vi "CONFIG PRES+TEMP+REG V115.vi"() -> ()   [LabVIEW 2022 SP3]
uses:
  Pressions/Gestion grappe/TypeDef_Seuil Jauge Pression_CN.ctl
  Enum/Enum conf 1.ctl
  Variables globales/Variable glob Edwards.vi
  Variables globales/Variable glob Th.vi
  Variables globales/Variable glob Pt.vi
  Variables globales/Variable glob Leybold.vi
  Variables globales/Variable glob Keller.vi
  Variables globales/Variable glob generale.vi
  Variables globales/Variables glob EUROTHERM.vi
  Variables globales/Variable globale compteurs.vi
  Variables globales/Variable glob mails.vi
  <vilib>/Utility/config.llb/NI_LVConfig.lvlib
panel:
  in  "annuler":bool
  out "Dossier DATA local :":path
  in  "Commande onglet":T1(tab)=enum."THERMOCOUPLES"
  in  "Domaine envoi mail":string
  in  "Serveur sortant":string
  in  "Domaine mail labo":string
  in  "Noms personnels station":string[](array[string])
  in  "NOMS DES CENTER ONE":string[](array[string])
  in  "Nb LEYBOLD":i8 caption="Nombre de coffrets LEYBOLD" min=0 max=20
  in  "Ports COM LEYBOLDS":refnum<visa-resource-name>[](array[refnum])
  in  "Nb EDWARDS":i8 caption="Nombre de coffrets EDWARDS" min=0 max=20
  in  "Ports COM EDWARDS":refnum<visa-resource-name>[](array[refnum])
  in  "Voies EDWARDS":u8[][](array[numeric])=[[1, 1], [1, 0]] max=6
  in  "Noms jauges":string[][](array[string])
  in  "Seuil Jauge":T2={"Descente en Pression"={"Min Mesure Piezo"=5.0, "Min Mesure Pirani"=0.0002}, "Montée en Pression"={"Max Mesure Pirani"=10.0, "Max Mesure Penning"=0.0004}} {"Montée en Pression"."Max Mesure Penning" format="%.2e"; "Montée en Pression"."Max Mesure Pirani" format="%.2e"; "Descente en Pression"."Min Mesure Pirani" format="%.2e"; "Descente en Pression"."Min Mesure Piezo" format="%.2e"}
  in  "Nombre de grappes":u8
  in  "Noms grappes":string[](array[string])
  in  "Grappes":u16[][](array[ring]) items=["GAZ TIC 1", "GAZ TIC 2", "GAZ TIC 3", "GAZ TIC 4", "GAZ TIC 5", "GAZ TIC 6", "SUV Ptu 1", "SUV Ptu 2", "SUV Ptu 3", "SUV Ptu 4", "SUV Ptu 5", "SUV Ptu 6", "SUV TIC 1", "SUV TIC 2", "SUV TIC 3", "SUV TIC 4", "SUV TIC 5", "SUV TIC 6", "MIR Ptu 1", "MIR  Ptu 2", "MIR  Ptu 3", "MIR  Ptu 4", "MIR  Ptu 5", "MIR  Ptu 6", "MIR TIC 1", "MIR TIC 2 ", "MIR TIC 3 ", "MIR TIC 4", "MIR TIC 5", "MIR TIC 6 ", "MON Ptu 1", "MON Ptu 2", "MON Ptu 3", "MON Ptu 4", "MON Ptu 5", "MON Ptu 6", "MON TIC 1", "MON TIC 2", "MON TIC 3", "MON TIC 4", "MON TIC 5", "MON TIC 6", "REF TIC 1", "REF TIC 2", "REF TIC 3", "REF TIC 4", "REF TIC 5", "REF TIC 6", "REF Ptu 1", "REF Ptu 2", "REF Ptu 3", "REF Ptu 4", "REF Ptu 5", "REF Ptu 6"]
  in  "Noms taches Th":refnum<k21>[](array[refnum]) caption="Noms des taches associees aux modules"
  in  "Nombre de tâches thermocouples":u8
  in  "NB Th par tâche":i16[](array[numeric]) caption="Nombre de Th par tâche"
  in  "Nombre de tâches Pt":u8
  in  "Noms taches Pt":refnum<k21>[](array[refnum]) caption="Noms des taches associees aux modules"
  in  "NB Pt par tâche":i16[](array[numeric]) caption="Nombre de Pt par tâche"
  in  "sur port COM :":u16(ring) items=["COM6"]
  in  "Nb COM REG":u8 caption="Nombre de port COM"
  in  "Nb reg":u8[](array[numeric]) caption="Nombre de regulateurs" max=6 step=1
  in  "Ports COM REG":refnum<visa-resource-name>[](array[refnum]) caption="Ports COM"
  in  "Regulateurs EUROTHERM":T3(array[cluster])
  in  "Port COM KELLER":refnum<visa-resource-name>="COM7"
  in  "Nb KELLER":i32 caption="Nombre de capteurs KELLER" min=0 max=20
  in  "Adresses KELLER":i16[](array[numeric])=[1, 1]
  in  "Noms capteurs KELLER":string[](array[string])
  in  "Nb compteurs":u8 caption="Nombre de compteurs" max=8
  in  "Noms des compteurs":string[](array[string])
  in  "Nom tache compteurs":refnum<k21> caption="Nom de la tache associee aux compteurs"
  in  "Nom cuve":u16(ring) caption="Nom du simulateur spatial :" items=["", "JUPITER", "MARS", "MERCURE", "NEPTUNE", "PLUTON", "SATURNE", "SUN", "TERRE", "URANUS", "VENUS", "LUV"]
  in  "stop":bool
  # "CONFIGURATION matérielle pour\nlES ACQUISITIONS instrumentation"
  # "Ce logiciel et les informations qu'il contient, sont la propriété de l’IAS et ne peuvent être diffusés sans l’autorisation de la Station d’étalonnage"
  # "Capacitive ou Piezo"
  # "Pirani"
  # "Penning"
  # "THERMOCOUPLES"
  # "REMARQUE :\nLes \"Paramètres de cadencement\" configures dans MAX\ndoivent être definis aux valeurs ci-dessous"
  # "Platines 100 ohm"
  # "REMARQUE :\nLes \"Paramètres de cadencement\" configures dans MAX\ndoivent être definis aux valeurs ci-dessous"
  # "RÉGULATEURS EUROTHERM"
  # "KELLER"
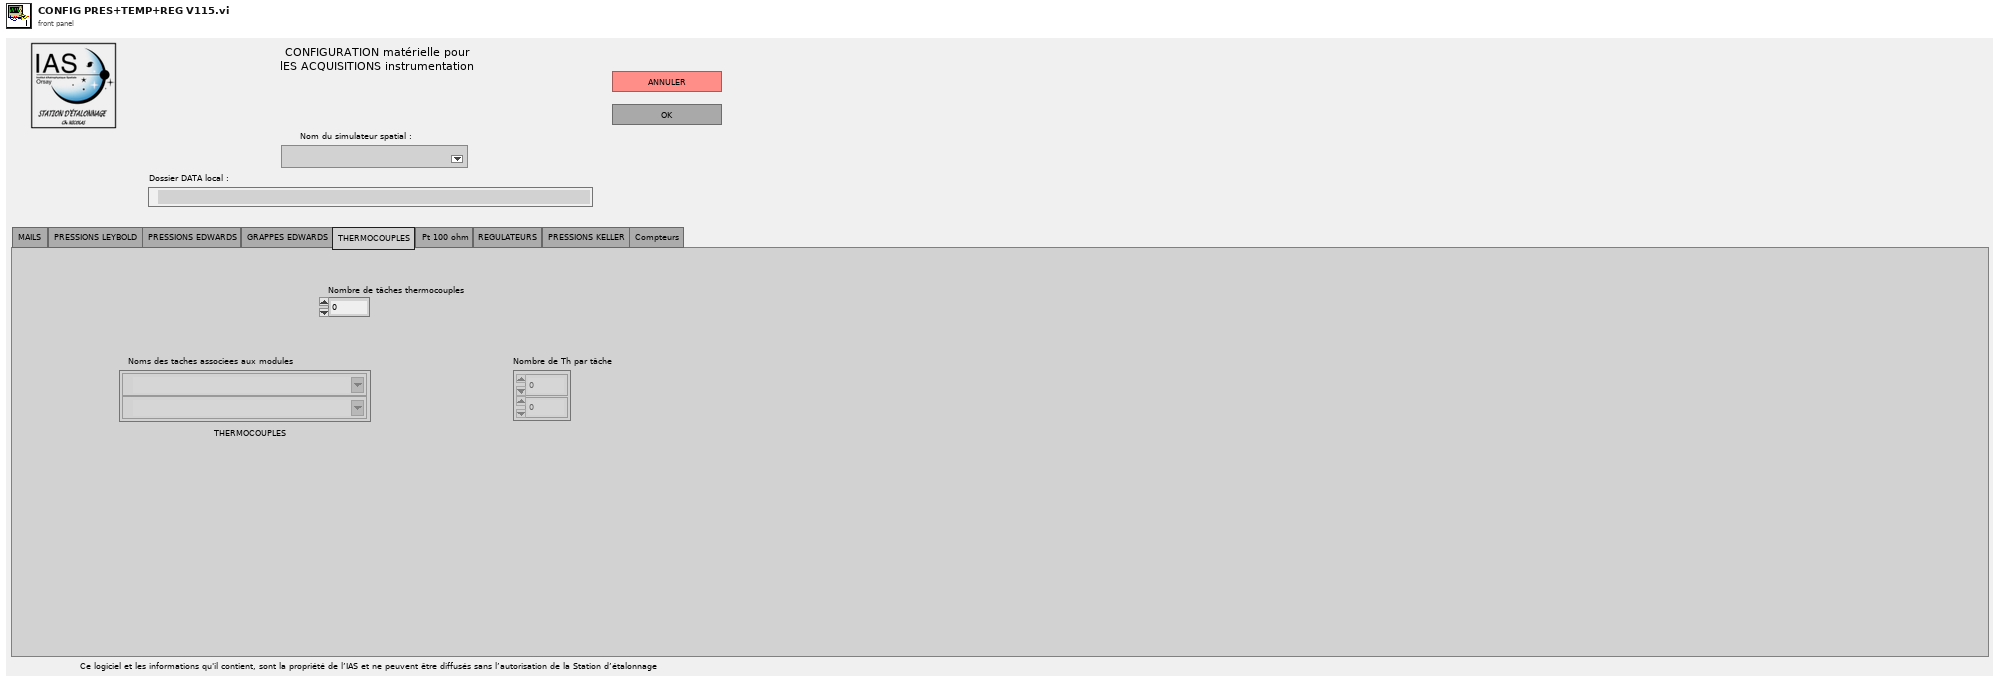
[diagram p1: front panel]
types:
  T1 = enum32{"MAILS", "PRESSIONS LEYBOLD", "PRESSIONS EDWARDS", "GRAPPES EDWARDS", "THERMOCOUPLES", "Pt 100 ohm ", "REGULATEURS", "PRESSIONS KELLER", "Compteurs"}
  T2 = typedef "TypeDef_Seuil Jauge Pression_CN.ctl" = cluster{"Descente en Pression":cluster{"Min Mesure Piezo":dbl, "Min Mesure Pirani":dbl}, "Montée en Pression":cluster{"Max Mesure Pirani":dbl, "Max Mesure Penning":dbl}}
  T3 = cluster{"1 COM reg":cluster{"Nom":string, "Adresse":u8}[]}[]
  T4 = typedef "Enum conf 1.ctl" = enum16{"init", "ouvrir fichier config", "init var locales 1", "init var locales 2", "init var locales 3", "choix operateur", "enregistrer fichier config", "annule", "fin"}
  T5 = cluster{"Rég EUROTHERM 2":cluster{"Nom":string, "Adresse":u8}[]}
  T6 = enum8{"Enabled", "Disabled", "Disabled and Grayed Out"}
  T7 = typedef "NI_LVConfig.lvlib/Config Data RefNum.ctl" = refnum<k1>
  T8 = cluster{"Nom tache Pt":refnum<k21>, "Noms des Pt":string[], "Nb Pt":i16, "Selection Pt":bool[], "Nom Pt selectionnees":string[]}[]
  T9 = cluster{"Nom tache Th":refnum<k21>, "Noms des Th":string[], "Nb Th":i16, "Selection Th":bool[], "Nom Th selectionnes":string[]}[]
  T10 = cluster{"Nom tache compteurs":refnum<k21>, "Noms des compteurs":string[], "Selection":bool[], "Init compteurs":dbl[], "Noms compteurs selectionnes":string[]}
  T11 = cluster{"1 COM reg":cluster{"Nom":string, "Adresse":u8}[]}
  T12 = cluster{"Nom tache Th":refnum<k21>, "Noms des Th":string[], "Nb Th":i16, "Selection Th":bool[], "Nom Th selectionnes":string[]}
  T13 = cluster{"Nom tache Pt":refnum<k21>, "Noms des Pt":string[], "Nb Pt":i16, "Selection Pt":bool[], "Nom Pt selectionnees":string[]}
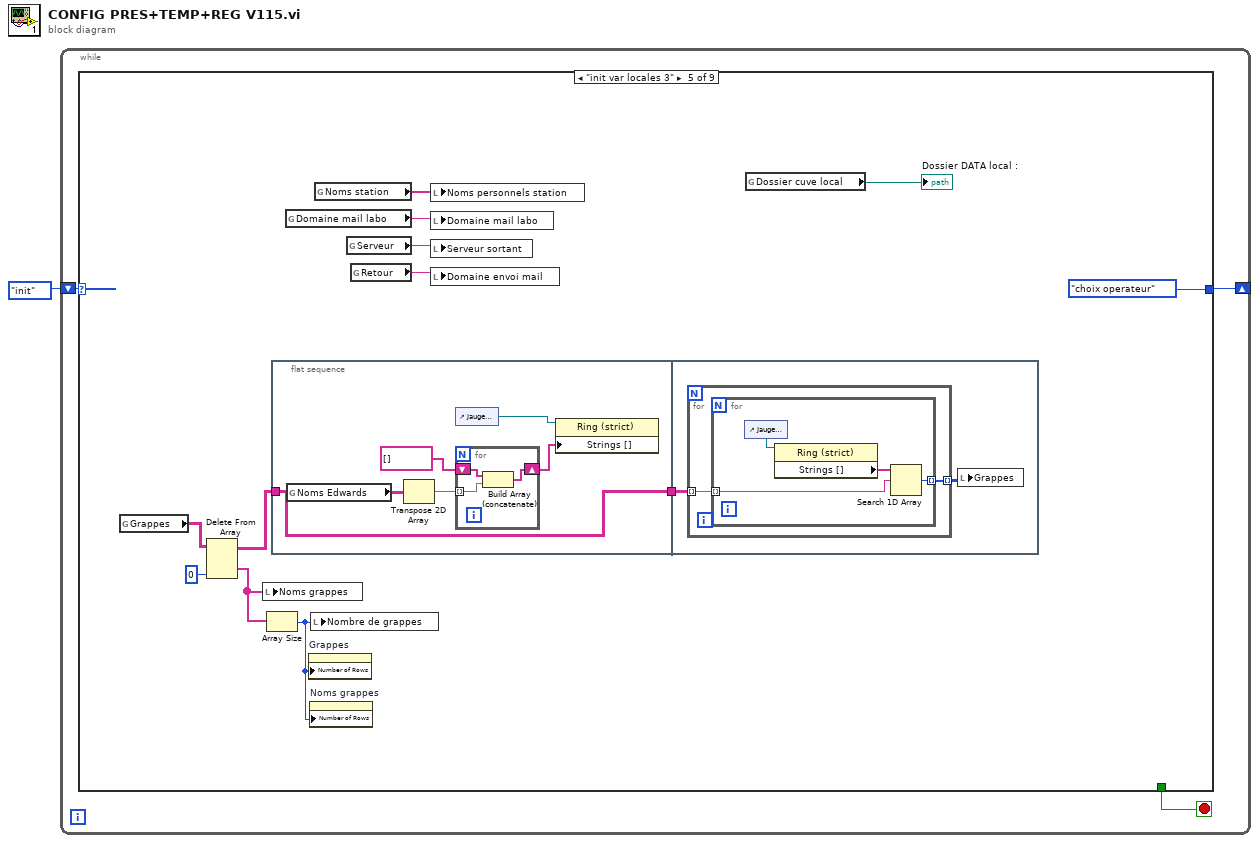
[diagram p0: block diagram]
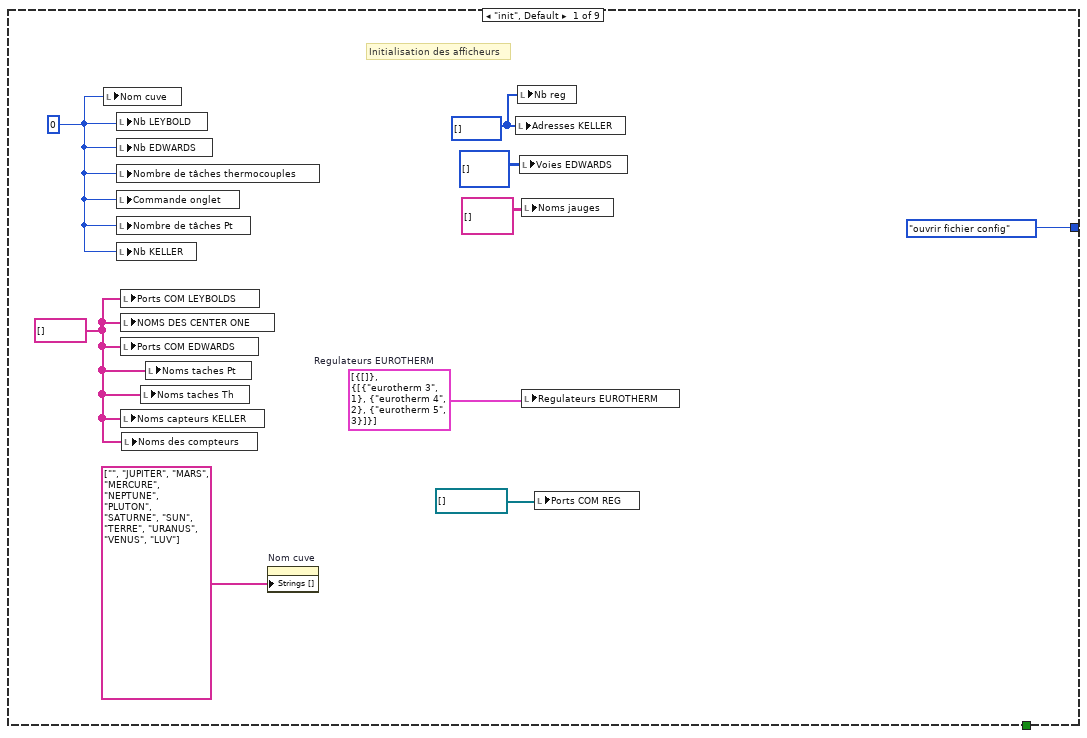
[diagram p2: hidden frame]
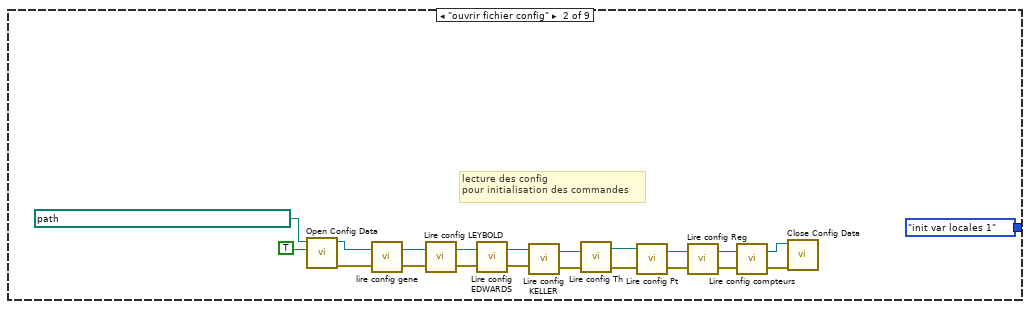
[diagram p3: hidden frame]
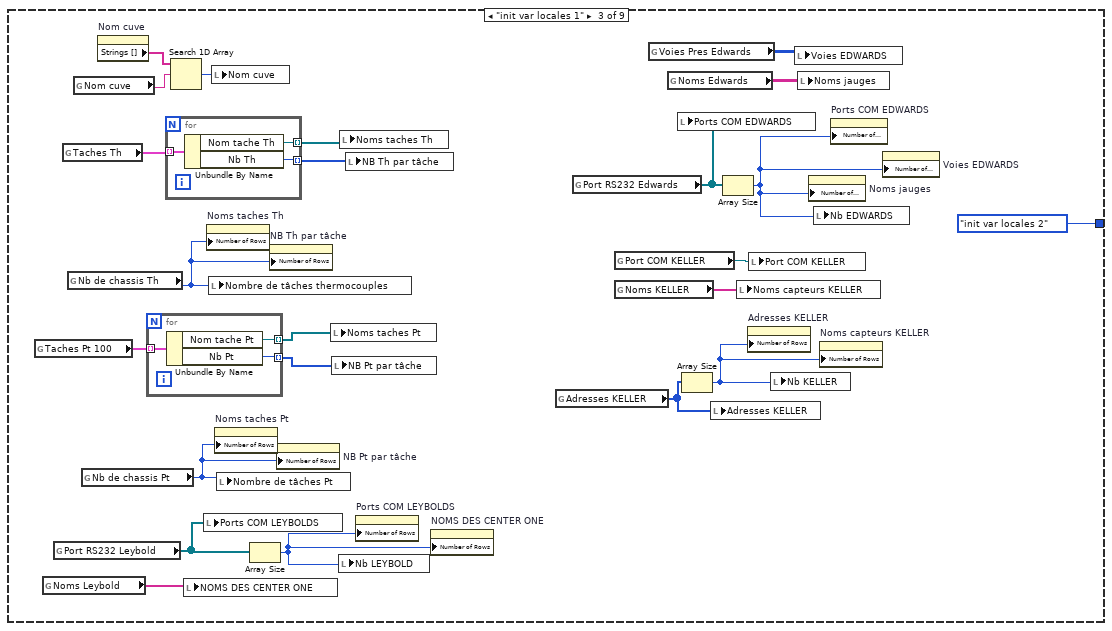
[diagram p4: hidden frame]
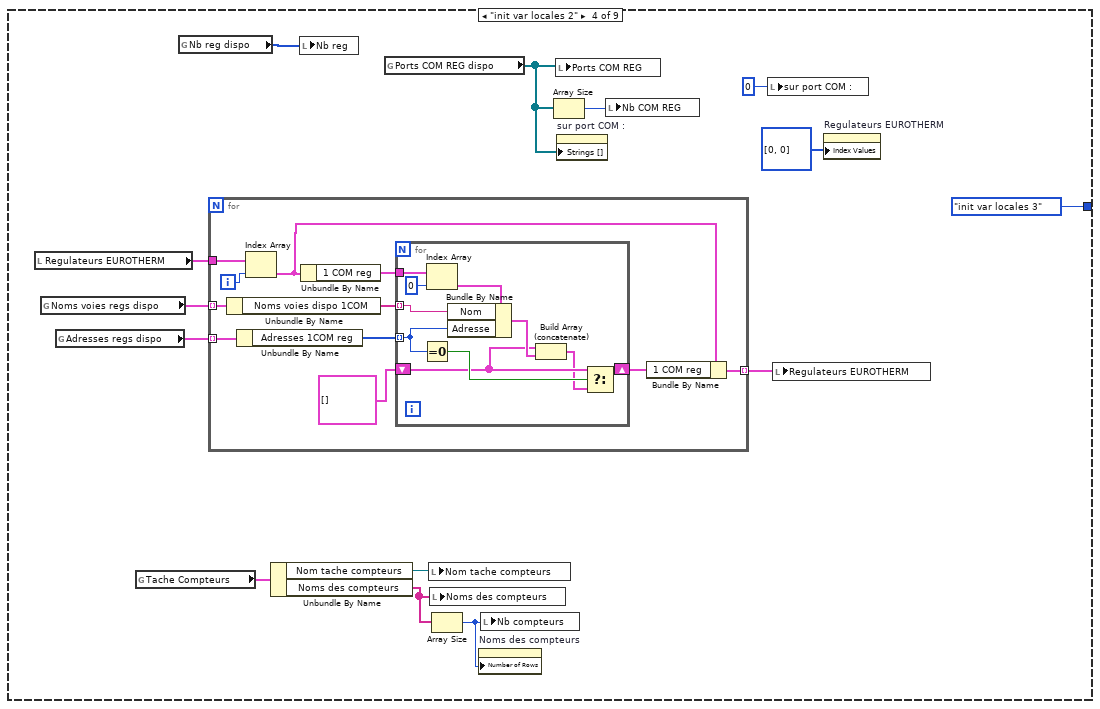
[diagram p5: hidden frame]
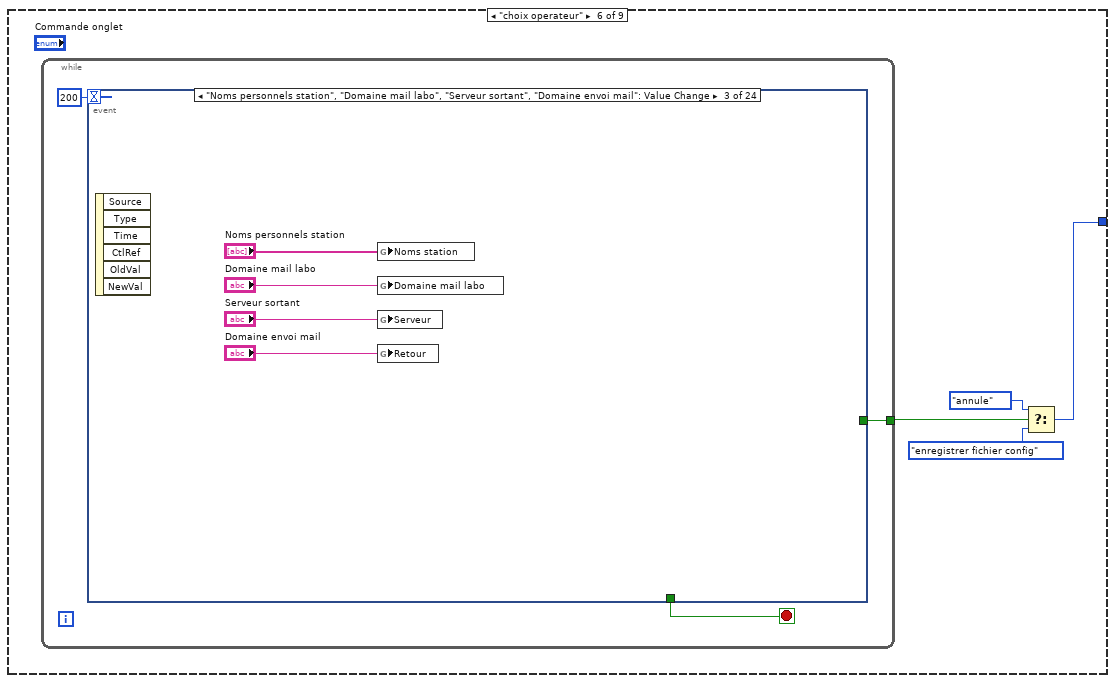
[diagram p6: hidden frame]
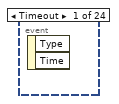
[diagram p7: hidden frame]
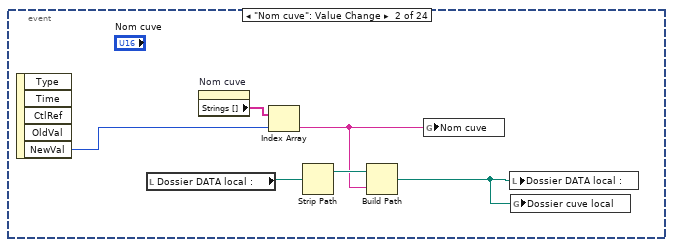
[diagram p8: hidden frame]
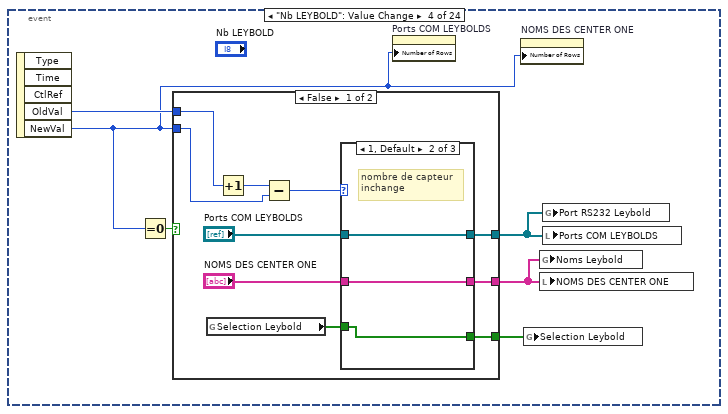
[diagram p9: hidden frame]
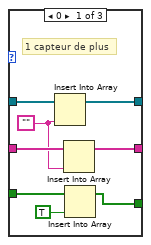
[diagram p10: hidden frame]
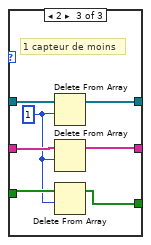
[diagram p11: hidden frame]
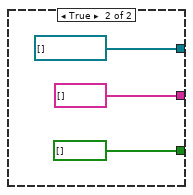
[diagram p12: hidden frame]
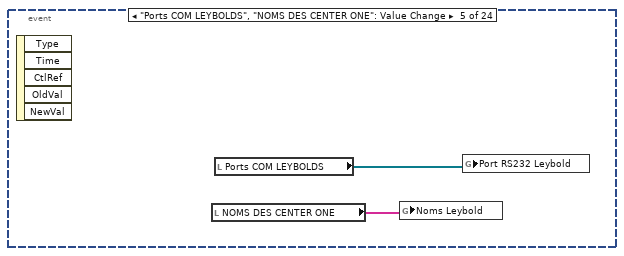
[diagram p13: hidden frame]
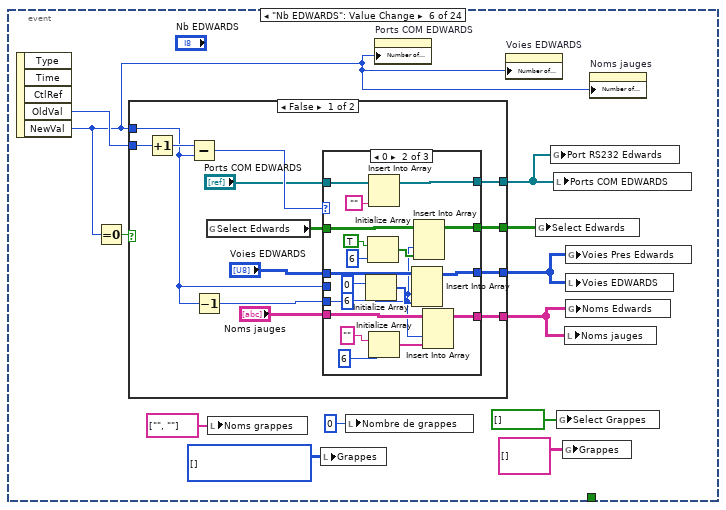
[diagram p14: hidden frame]
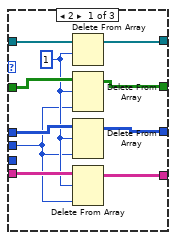
[diagram p15: hidden frame]
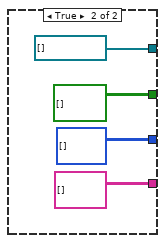
[diagram p17: hidden frame]
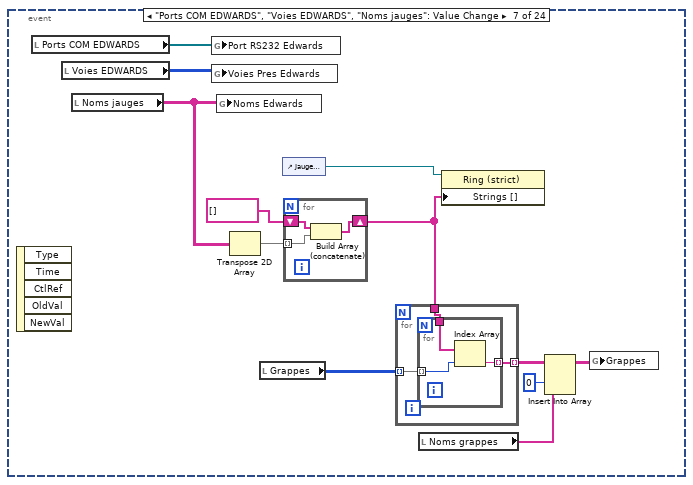
[diagram p18: hidden frame]
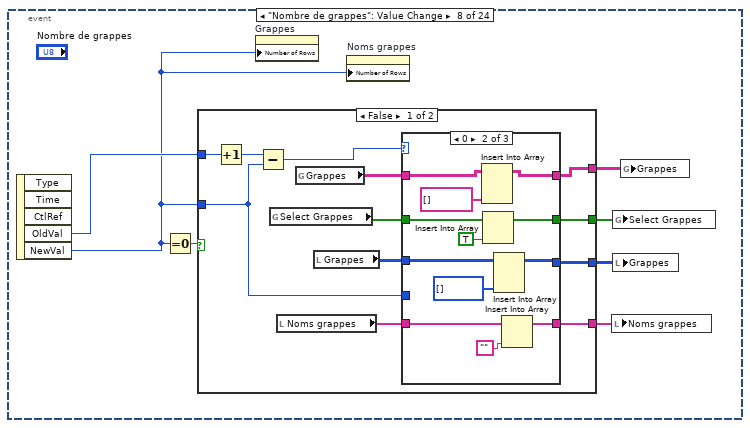
[diagram p19: hidden frame]
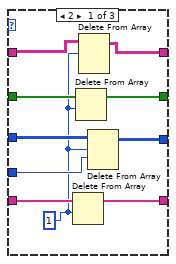
[diagram p20: hidden frame]
diagram:
  n1 = while {
    shift-right: [w3] -> _
    shift-left: Enum_conf_1."init" ("Énum") -> [w4]
    stop <- w2 stop-if-true
    n2 = case shown="\"init var locales 3\"" w4 {
      tunnel: [Enum_conf_1."ouvrir fichier config" ("Énum") Enum_conf_1."init var locales 1" ("Énum") Enum_conf_1."init var locales 2" ("Énum") Enum_conf_1."init var locales 3" ("Énum") Enum_conf_1."choix operateur" ("Énum") w128 Enum_conf_1."fin" ("Énum") Enum_conf_1."fin" ("Énum") Enum_conf_1."init" ("Énum")] -> w3
      tunnel: [_ _ _ _ _ _ _ _ TRUE] -> w2
      frame "init", Default {
        w6 = T3 [{"1 COM reg"=[]}, {"1 COM reg"=[{"Nom"="eurotherm 3", "Adresse"=1}, {"Nom"="eurotherm 4", "Adresse"=2}, {"Nom"="eurotherm 5", "Adresse"=3}]}]  # Regulateurs EUROTHERM
        w8 = i32[] [] ("Voies EDWARDS")
        w5 = string[] [] ("NOMS DES CENTER ONE")
        w9 = i8 0 ("Nombre de coffrets LEYBOLD")
        # "Initialisation des afficheurs"
        n3 = local write "Nom cuve"(w9) -> ()
        n4 = local write "Nb LEYBOLD"(w9) -> ()
        n5 = local write "Nb EDWARDS"(w9) -> ()
        n6 = local write "Nombre de tâches thermocouples"(w9) -> ()
        n7 = local write "Commande onglet"(w9) -> ()
        n8 = local write "Nombre de tâches Pt"(w9) -> ()
        n9 = local write "Nb KELLER"(w9) -> ()
        n10 = local write "Ports COM LEYBOLDS"(w5) -> ()
        n11 = local write "NOMS DES CENTER ONE"(w5) -> ()
        n12 = local write "Ports COM EDWARDS"(w5) -> ()
        n13 = local write "Noms capteurs KELLER"(w5) -> ()
        n14 = local write "Noms des compteurs"(w5) -> ()
        n15 = local write "Noms taches Th"(w5) -> ()
        n16 = local write "Noms taches Pt"(w5) -> ()
        n17 = property on="Nom cuve" class="Ring (strict)"("Strings []"=string[] ["", "JUPITER", "MARS", "MERCURE", "NEPTUNE", "PLUTON", "SATURNE", "SUN", "TERRE", "URANUS", "VENUS", "LUV"] ("Chaînes []")) -> ()  [unwired: 2 in, 2 out]
        n18 = local write "Adresses KELLER"(w8) -> ()
        n19 = local write "Nb reg"(w8) -> ()
        n20 = local write "Voies EDWARDS"(i32[][] [] ("Voies EDWARDS")) -> ()
        n21 = local write "Noms jauges"(string[][] [] ("Noms jauges")) -> ()
        n22 = local write "Regulateurs EUROTHERM"(w6) -> ()
        n23 = local write "Ports COM REG"(refnum<visa-resource-name>[] [] ("Ports COM")) -> ()
      }
      frame "ouvrir fichier config" {
        # "lecture des config \npour initialisation des commandes"
        n24 = call <vilib>:"Open Config Data.vi"("create file if necessary (T)"=TRUE ("create file if necessary? (T)"), "configuration file path"=path "C:/LABVIEW/PRES+TEMP+REG dernière version/Configurations/config acqui.ini") -> ("error out"=w27:errorcluster, "refnum"=w25:T7)  [unwired: 7 in, 1 out]
        n25 = call "lire config gene.vi"("error in"=w27, "refnum"=w25) -> ("error out"=w26:errorcluster, "refnum out"=w24:T7)
        n26 = call "Lire config LEYBOLD.vi"("error in (no error)"=w26, "refnum"=w24) -> ("error out"=w32:errorcluster, "refnum out"=w23:T7)
        n27 = call "Lire config EDWARDS.vi"("error in (no error)"=w32, "refnum"=w23) -> ("error out"=w30:errorcluster, "refnum out"=w22:T7)
        n28 = call "Lire config KELLER.vi"("error in (no error)"=w30, "refnum"=w22) -> ("error out"=w29:errorcluster, "refnum out"=w21:T7)
        n29 = call "Lire config Th.vi"("error in (no error)"=w29, "refnum"=w21) -> ("error out"=w28:errorcluster, "refnum out"=w20:T7)
        n30 = call "Lire config Pt.vi"("error in (no error)"=w28, "refnum"=w20) -> ("error out"=w18:errorcluster, "refnum out"=w19:T7)
        n31 = call "Lire config Reg.vi"("error in (no error)"=w18, "refnum"=w19) -> ("error out"=w15:errorcluster, "refnum out"=w17:T7)
        n32 = call "Lire config compteurs.vi"("error in"=w15, "refnum"=w17) -> ("error out"=w14:errorcluster, "refnum out"=w16:T7)
        n33 = call <vilib>:"Close Config Data.vi"("error in (no error)"=w14, "refnum"=w16) -> ()  [unwired: 8 in, 2 out]
      }
      frame "init var locales 1" {
        n34 = global read "Variable glob Pt.vi" "Taches Pt 100"() -> (w40:T8)
        n35 = global read "Variable glob Leybold.vi" "Noms Leybold"() -> (w54:string[])
        n36 = global read "Variable glob Leybold.vi" "Port RS232 Leybold"() -> (w55:refnum<visa-resource-name>[])
        n37 = global read "Variable glob Th.vi" "Taches Th"() -> (w37:T9)
        n38 = global read "Variable glob Th.vi" "Nb de chassis Th"() -> (w47:u8)
        n39 = global read "Variable glob generale.vi" "Nom cuve"() -> (w41:string)
        n40 = global read "Variable glob Pt.vi" "Nb de chassis Pt"() -> (w46:u8)
        n41 = property on="Nom cuve" class="Ring (strict)"() -> ("Strings []"=w43:string[])  [unwired: 2 in, 2 out]
        n42 = for {
          tunnel: w40 -> [w63] mode=indexing
          tunnel: [w62] -> w39 mode=indexing
          tunnel: [w61] -> w38 mode=indexing
          n43 = Unbundle By Name(w63) -> ("Nom tache Pt"=w62:refnum<k21>, "Nb Pt"=w61:i16)
        }
        n44 = for {
          tunnel: w37 -> [w60] mode=indexing
          tunnel: [w59] -> w36 mode=indexing
          tunnel: [w58] -> w35 mode=indexing
          n45 = Unbundle By Name(w60) -> ("Nom tache Th"=w59:refnum<k21>, "Nb Th"=w58:i16)
        }
        n46 = Search 1D Array(1D array=w43, element=w41) -> (index of element=w42:i32)  [unwired: 1 in]
        n47 = local write "NOMS DES CENTER ONE"(w54) -> ()
        n48 = local write "Ports COM LEYBOLDS"(w55) -> ()
        n49 = property on="Noms taches Th" class="Arr (strict)"("Number of Rows"=w47) -> ()  [unwired: 2 in, 2 out]
        n50 = local write "Nombre de tâches thermocouples"(w47) -> ()
        n51 = local write "Nom cuve"(w42) -> ()
        n52 = property on="Noms taches Pt" class="Arr (strict)"("Number of Rows"=w46) -> ()  [unwired: 2 in, 2 out]
        n53 = local write "Nombre de tâches Pt"(w46) -> ()
        n54 = Array Size(array=w55) -> (size(s)=w50:i32)
        n55 = property on="NB Th par tâche" class="Arr (strict)"("Number of Rows"=w47) -> ()  [unwired: 2 in, 2 out]
        n56 = property on="NB Pt par tâche" class="Arr (strict)"("Number of Rows"=w46) -> ()  [unwired: 2 in, 2 out]
        n57 = local write "Noms taches Pt"(w39) -> ()
        n58 = local write "NB Pt par tâche"(w38) -> ()
        n59 = local write "Nb LEYBOLD"(w50) -> ()
        n60 = local write "Noms taches Th"(w36) -> ()
        n61 = local write "NB Th par tâche"(w35) -> ()
        n62 = property on="Ports COM LEYBOLDS" class="Arr (strict)"("Number of Rows"=w50) -> ()  [unwired: 2 in, 2 out]
        n63 = property on="NOMS DES CENTER ONE" class="Arr (strict)"("Number of Rows"=w50) -> ()  [unwired: 2 in, 2 out]
        n64 = global read "Variable glob Keller.vi" "Adresses KELLER"() -> (w52:i16[])
        n65 = global read "Variable glob Edwards.vi" "Port RS232 Edwards"() -> (w56:refnum<visa-resource-name>[])
        n66 = global read "Variable glob Keller.vi" "Port COM KELLER"() -> (w53:refnum<visa-resource-name>)
        n67 = global read "Variable glob Keller.vi" "Noms KELLER"() -> (w51:string[])
        n68 = global read "Variable glob Edwards.vi" "Voies Pres Edwards"() -> (w57:i8[][])
        n69 = global read "Variable glob Edwards.vi" "Noms Edwards"() -> (w45:string[][])
        n70 = local write "Ports COM EDWARDS"(w56) -> ()
        n71 = Array Size(array=w52) -> (size(s)=w48:i32)
        n72 = local write "Adresses KELLER"(w52) -> ()
        n73 = Array Size(array=w56) -> (size(s)=w49:i32)
        n74 = local write "Noms capteurs KELLER"(w51) -> ()
        n75 = property on="Adresses KELLER" class="Arr (strict)"("Number of Rows"=w48) -> ()  [unwired: 2 in, 2 out]
        n76 = local write "Port COM KELLER"(w53) -> ()
        n77 = local write "Nb KELLER"(w48) -> ()
        n78 = local write "Voies EDWARDS"(w57) -> ()
        n79 = local write "Noms jauges"(w45) -> ()
        n80 = property on="Noms jauges" class="Arr (strict)"("Number of Columns"=w49) -> ()  [unwired: 2 in, 2 out]
        n81 = local write "Nb EDWARDS"(w49) -> ()
        n82 = property on="Noms capteurs KELLER" class="Arr (strict)"("Number of Rows"=w48) -> ()  [unwired: 2 in, 2 out]
        n83 = property on="Ports COM EDWARDS" class="Arr (strict)"("Number of Columns"=w49) -> ()  [unwired: 2 in, 2 out]
        n84 = property on="Voies EDWARDS" class="Arr (strict)"("Number of Columns"=w49) -> ()  [unwired: 2 in, 2 out]
      }
      frame "init var locales 2" {
        n85 = local read "Regulateurs EUROTHERM"() -> (w69:T3)
        n86 = global read "Variables glob EUROTHERM.vi" "Noms voies regs dispo"() -> (w71:cluster{"Noms voies dispo 1COM":string[]}[])
        n87 = global read "Variables glob EUROTHERM.vi" "Adresses regs dispo"() -> (w70:cluster{"Adresses 1COM reg":u16[]}[])
        n88 = global read "Variable globale compteurs.vi" "Tache Compteurs"() -> (w67:T10)
        n89 = global read "Variables glob EUROTHERM.vi" "Nb reg dispo"() -> (w76:u8[])
        n90 = for {
          tunnel: w71 -> [w79] mode=indexing
          tunnel: w70 -> [w81] mode=indexing
          tunnel: w69 -> [w86]
          tunnel: [w87] -> w68 mode=indexing
          i -> [w84]
          n91 = Unbundle By Name(w79) -> ("Noms voies dispo 1COM"=w78:string[])
          n92 = Unbundle By Name(w81) -> ("Adresses 1COM reg"=w80:u16[])
          n93 = Index Array(array=w86, index=w84) -> (element=w85:T11)
          n94 = Unbundle By Name(w85) -> ("1 COM reg"=w88:cluster{"Nom":string, "Adresse":u8}[])
          n95 = for {
            tunnel: w88 -> [w97]
            tunnel: w78 -> [w98] mode=indexing
            tunnel: w80 -> [w93] mode=indexing
            shift-right: [w89] -> w83
            shift-left: cluster{"Nom":string, "Adresse":u8}[] [] -> [w91]
            n96 = Equal To 0?(x=w93) -> (x = 0?=w92:bool)
            n97 = Index Array(array=w97, index=0 ("indice")) -> (element=w95:cluster{"Nom":string, "Adresse":u8})
            n98 = Bundle By Name(cluster=w95, "Nom"=w98, "Adresse"=w93) -> (w94:cluster{"Nom":string, "Adresse":u8})
            n99 = Build Array (concatenate)(w91, w94) -> (w90:cluster{"Nom":string, "Adresse":u8}[])
            n100 = Select(t=w91, s=w92, f=w90) -> (s? t:f=w89:cluster{"Nom":string, "Adresse":u8}[])
          }
          n101 = Bundle By Name(cluster=w85, "1 COM reg"=w83) -> (w87:T11)
        }
        n102 = Unbundle By Name(w67) -> ("Nom tache compteurs"=w66:refnum<k21>, "Noms des compteurs"=w65:string[])
        n103 = local write "Nb reg"(w76) -> ()
        n104 = global read "Variables glob EUROTHERM.vi" "Ports COM REG dispo"() -> (w74:refnum<visa-resource-name>[])
        n105 = local write "Nom tache compteurs"(w66) -> ()
        n106 = local write "Noms des compteurs"(w65) -> ()
        n107 = Array Size(array=w65) -> (size(s)=w64:i32)
        n108 = property on="Noms des compteurs" class="Arr (strict)"("Number of Rows"=w64) -> ()  [unwired: 2 in, 2 out]
        n109 = local write "Nb compteurs"(w64) -> ()
        n110 = Array Size(array=w74) -> (size(s)=w75:i32)
        n111 = local write "Ports COM REG"(w74) -> ()
        n112 = property on="sur port COM :" class="Ring (strict)"("Strings []"=w74) -> ()  [unwired: 2 in, 2 out]
        n113 = local write "Nb COM REG"(w75) -> ()
        n114 = local write "sur port COM :"(u16 0) -> ()
        n115 = local write "Regulateurs EUROTHERM"(w68) -> ()
        n116 = property on="Regulateurs EUROTHERM" class="Arr (strict)"("Index Values"=u32[] [0, 0] ("Valeurs d'indice")) -> ()  [unwired: 2 in, 2 out]
      }
      frame "init var locales 3" {
        n117 = global read "Variable glob Edwards.vi" "Grappes"() -> (w108:string[][])
        n118 = Delete From Array(array=w108, index (col)=0 ("indice désactivé (col)")) -> (deleted portion=w106:string[], array with subset deleted=w109:string[][])  [unwired: 2 in]
        n119 = local write "Noms grappes"(w106) -> ()
        n120 = Array Size(array=w106) -> (size(s)=w105:i32)
        n121 = flat-sequence {
          tunnel: w109 -> [w111]
          tunnel: [w111] -> w103
          tunnel: w103 -> [w121]
          frame #0 {
            n122 = global read "Variable glob Edwards.vi" "Noms Edwards"() -> (w116:string[][])
            n123 = Transpose 2D Array(2D array=w116) -> (transposed array=w115:string[][])
            n124 = control-ref of="Jauge Grappe"() -> (w112:refnum<vi>)
            n125 = for {
              tunnel: w115 -> [w119] mode=indexing
              shift-right: [w117] -> w113
              shift-left: string[] [] -> [w118]
              n126 = Build Array (concatenate)(w118, w119) -> (w117:string[])
            }
            n127 = property class="Ring (strict)"(reference=w112, "Strings []"=w113) -> ()  [unwired: 1 in, 2 out]
          }
          frame #1 {
            n128 = for {
              tunnel: w121 -> [w123] mode=indexing
              tunnel: [w122] -> w120 mode=indexing
              n129 = for {
                tunnel: w123 -> [w127] mode=indexing
                tunnel: [w126] -> w122 mode=indexing
                n130 = control-ref of="Jauge Grappe"() -> (w125:refnum<vi>)
                n131 = property class="Ring (strict)"(reference=w125) -> ("Strings []"=w124:string[])  [unwired: 1 in, 2 out]
                n132 = Search 1D Array(1D array=w124, element=w127) -> (index of element=w126:i32)  [unwired: 1 in]
              }
            }
            n133 = local write "Grappes"(w120) -> ()
          }
        }
        n134 = global read "Variable glob mails.vi" "Domaine mail labo"() -> (w101:string)
        n135 = property on="Grappes" class="Arr (strict)"("Number of Rows"=w105) -> ()  [unwired: 2 in, 2 out]
        n136 = property on="Noms grappes" class="Arr (strict)"("Number of Rows"=w105) -> ()  [unwired: 2 in, 2 out]
        n137 = local write "Nombre de grappes"(w105) -> ()
        n138 = global read "Variable glob mails.vi" "Noms station"() -> (w102:string[])
        n139 = global read "Variable glob mails.vi" "Serveur"() -> (w100:string)
        n140 = global read "Variable glob mails.vi" "Retour"() -> (w99:string)
        n141 = local write "Noms personnels station"(w102) -> ()
        n142 = local write "Domaine mail labo"(w101) -> ()
        n143 = local write "Serveur sortant"(w100) -> ()
        n144 = local write "Domaine envoi mail"(w99) -> ()
        n145 = global read "Variable glob generale.vi" "Dossier cuve local"() -> (→"Dossier DATA local :":path)
      }
      frame "choix operateur" {
        n146 = while {
          tunnel: [w133] -> w131
          stop <- w132 stop-if-true
          n147 = event shown="[2] \"Noms personnels station\", \"Domaine mail labo\", \"Serveur sortant\", \"Domaine envoi mail\": Value Change" {
            selector: _ -> [_ _ _ _ _ _ _ _ _ _ _ _ _ _ _ _ _ _ _ _ _ _ _ _]
            dyn-events: _ -> [_ _ _ _ _ _ _ _ _ _ _ _ _ _ _ _ _ _ _ _ _ _ _ _]
            timeout: u32 200 ("attente (ms)") -> [_ _ _ _ _ _ _ _ _ _ _ _ _ _ _ _ _ _ _ _ _ _ _ _]
            tunnel: [_ _ _ _ _ _ _ _ _ _ _ _ _ _ _ _ _ _ _ _ _ _ "annuler" _] -> w133
            tunnel: [_ _ _ _ _ _ _ _ _ _ _ _ _ _ _ _ _ _ _ _ _ _ "annuler" "stop"] -> w132
            event Timeout {
              n148 = event-data() -> ()  [unwired: 1 in, 2 out]
            }
            event "Nom cuve": Value Change {
              n149 = event-data() -> ("NewVal"=w135:u16)  [unwired: 1 in, 4 out]
              n150 = local read "Dossier DATA local :"() -> (w138:path)
              n151 = property on="Nom cuve" class="Ring (strict)"() -> ("Strings []"=w140:string[])  [unwired: 2 in, 2 out]
              n152 = Index Array(array=w140, index=w135) -> (element=w136:string)
              n153 = Strip Path(path=w138) -> (stripped path=w137:path)  [unwired: 1 out]
              n154 = Build Path(base path=w137, name or relative path=w136) -> (appended path=w139:path)
              n155 = global write "Variable glob generale.vi" "Nom cuve"(w136) -> ()
              n156 = local write "Dossier DATA local :"(w139) -> ()
              n157 = global write "Variable glob generale.vi" "Dossier cuve local"(w139) -> ()
            }
            event "Noms personnels station", "Domaine mail labo", "Serveur sortant", "Domaine envoi mail": Value Change {
              n158 = event-data() -> ()  [unwired: 1 in, 6 out]
              n159 = global write "Variable glob mails.vi" "Noms station"("Noms personnels station") -> ()
              n160 = global write "Variable glob mails.vi" "Domaine mail labo"("Domaine mail labo") -> ()
              n161 = global write "Variable glob mails.vi" "Serveur"("Serveur sortant") -> ()
              n162 = global write "Variable glob mails.vi" "Retour"("Domaine envoi mail") -> ()
            }
            event "Nb LEYBOLD": Value Change {
              n163 = event-data() -> ("OldVal"=w150:i8, "NewVal"=w145:i8)  [unwired: 1 in, 3 out]
              n164 = Equal To 0?(x=w145) -> (x = 0?=w146:bool)
              n165 = case shown="False" w146 {
                tunnel: w150 -> [w158 _]
                tunnel: w145 -> [w157 _]
                tunnel: [w155 bool[] [] ("Sélection Leybold")] -> w149
                tunnel: [w154 refnum<visa-resource-name>[] [] ("Ports COM LEYBOLDS")] -> w148
                tunnel: [w153 string[] [] ("NOMS DES CENTER ONE")] -> w147
                frame False {
                  n166 = global read "Variable glob Leybold.vi" "Selection Leybold"() -> (w156:bool[])
                  n167 = Increment(x=w158) -> (x+1=w160:i8)
                  n168 = Subtract(x=w160, y=w157) -> (x-y=w159:i8)
                  n169 = case shown="1, Default" w159 {
                    tunnel: "Ports COM LEYBOLDS" -> [w168 w170 w178]
                    tunnel: "NOMS DES CENTER ONE" -> [w166 w169 w177]
                    tunnel: [w167 w170 w176] -> w154
                    tunnel: [w165 w169 w175] -> w153
                    tunnel: w156 -> [w164 w171 w174]
                    tunnel: [w162 w171 w172] -> w155
                    frame 0 {
                      w161 = ""
                      # "1 capteur de plus"
                      n170 = Insert Into Array(array=w168, new element=w161) -> (w167:refnum<visa-resource-name>[])  [unwired: 1 in]
                      n171 = Insert Into Array(array=w166, new element=w161) -> (w165:string[])  [unwired: 1 in]
                      n172 = Insert Into Array(array=w164, new element=TRUE) -> (w162:bool[])  [unwired: 1 in]
                    }
                    frame 1, Default {
                      # "nombre de capteur\ninchange"
                    }
                    frame 2 {
                      w173 = 1 ("longueur")
                      # "1 capteur de moins"
                      n173 = Delete From Array(array=w178, length=w173) -> (array with subset deleted=w176:refnum<visa-resource-name>[])  [unwired: 1 in, 1 out]
                      n174 = Delete From Array(array=w177, length=w173) -> (array with subset deleted=w175:string[])  [unwired: 1 in, 1 out]
                      n175 = Delete From Array(array=w174, length=w173) -> (array with subset deleted=w172:bool[])  [unwired: 1 in, 1 out]
                    }
                  }
                }
                frame True {
                }
              }
              n176 = property on="Ports COM LEYBOLDS" class="Arr (strict)"("Number of Rows"=w145) -> ()  [unwired: 2 in, 2 out]
              n177 = property on="NOMS DES CENTER ONE" class="Arr (strict)"("Number of Rows"=w145) -> ()  [unwired: 2 in, 2 out]
              n178 = global write "Variable glob Leybold.vi" "Selection Leybold"(w149) -> ()
              n179 = global write "Variable glob Leybold.vi" "Noms Leybold"(w147) -> ()
              n180 = local write "NOMS DES CENTER ONE"(w147) -> ()
              n181 = global write "Variable glob Leybold.vi" "Port RS232 Leybold"(w148) -> ()
              n182 = local write "Ports COM LEYBOLDS"(w148) -> ()
            }
            event "Ports COM LEYBOLDS", "NOMS DES CENTER ONE": Value Change {
              n183 = event-data() -> ()  [unwired: 1 in, 5 out]
              n184 = local read "NOMS DES CENTER ONE"() -> (w182:string[])
              n185 = local read "Ports COM LEYBOLDS"() -> (w183:refnum<visa-resource-name>[])
              n186 = global write "Variable glob Leybold.vi" "Noms Leybold"(w182) -> ()
              n187 = global write "Variable glob Leybold.vi" "Port RS232 Leybold"(w183) -> ()
            }
            event "Nb EDWARDS": Value Change {
              w184 = u16[][] [] items=["Piezo groupe", "Pirani groupe", "Penning groupe", "", "", "", "Penning RGA", "Pirani RGA", "Pirani pompage RGA", "", "", ""] ("Grappes")
              n188 = event-data() -> ("OldVal"=w195:i8, "NewVal"=w189:i8)  [unwired: 1 in, 3 out]
              n189 = Equal To 0?(x=w189) -> (x = 0?=w190:bool)
              n190 = case shown="False" w190 {
                tunnel: w195 -> [w205 _]
                tunnel: w189 -> [w204 _]
                tunnel: [w199 bool[][] [] ("Sélect Edwards")] -> w194
                tunnel: [w198 refnum<visa-resource-name>[] [] ("Ports COM EDWARDS")] -> w193
                tunnel: [w197 u8[][] [] ("Voies EDWARDS")] -> w192
                tunnel: [w196 string[][] [] ("Noms jauges")] -> w191
                frame False {
                  n191 = Increment(x=w205) -> (x+1=w207:i8)
                  n192 = Subtract(x=w207, y=w204) -> (x-y=w206:i8)
                  n193 = Decrement(x=w204) -> (x-1=w208:i8)
                  n194 = global read "Variable glob Edwards.vi" "Select Edwards"() -> (w200:bool[][])
                  n195 = case shown="0" w206 {
                    tunnel: "Ports COM EDWARDS" -> [w218 w237 w240]
                    tunnel: "Voies EDWARDS" -> [w216 w235 w238]
                    tunnel: [w217 w236 w240] -> w198
                    tunnel: [w215 w234 w238] -> w197
                    tunnel: "Noms jauges" -> [w214 w233 w239]
                    tunnel: [w213 w232 w239] -> w196
                    tunnel: w208 -> [_ w220 _]
                    tunnel: w204 -> [w210 _ _]
                    tunnel: w200 -> [w212 w225 w241]
                    tunnel: [w209 w224 w241] -> w199
                    frame 2 {
                      w211 = 1 ("longueur")
                      n196 = Delete From Array(array=w218, length=w211) -> (array with subset deleted=w217:refnum<visa-resource-name>[])  [unwired: 1 in, 1 out]
                      n197 = Delete From Array(array=w212, length=w211, index (col)=w210) -> (array with subset deleted=w209:bool[][])  [unwired: 1 in, 1 out]
                      n198 = Delete From Array(array=w216, length=w211, index (col)=w210) -> (array with subset deleted=w215:u8[][])  [unwired: 1 in, 1 out]
                      n199 = Delete From Array(array=w214, length=w211, index (col)=w210) -> (array with subset deleted=w213:string[][])  [unwired: 1 in, 1 out]
                    }
                    frame 0 {
                      n200 = Initialize Array(0 ("nouvel élément/sous-tableau"), 6 ("taille de la dimension")) -> (w228:i32[])
                      n201 = Initialize Array(TRUE, 6 ("taille de la dimension")) -> (w221:bool[])
                      n202 = Insert Into Array(array=w237, new element="") -> (w236:refnum<visa-resource-name>[])  [unwired: 1 in]
                      n203 = Initialize Array("", 6 ("taille de la dimension")) -> (w226:string[])
                      n204 = Insert Into Array(array=w235, index (col)=w220, new element=w228) -> (w234:u8[][])  [unwired: 1 in]
                      n205 = Insert Into Array(array=w225, index (col)=w220, new element=w221) -> (w224:bool[][])  [unwired: 1 in]
                      n206 = Insert Into Array(array=w233, index (col)=w220, new element=w226) -> (w232:string[][])  [unwired: 1 in]
                    }
                    frame 1, Default {
                    }
                  }
                }
                frame True {
                }
              }
              n207 = local write "Noms grappes"(string[] ["", ""] ("Noms grappes")) -> ()
              n208 = local write "Grappes"(w184) -> ()
              n209 = local write "Nombre de grappes"(u8 0 ("Nombre de grappes")) -> ()
              n210 = property on="Ports COM EDWARDS" class="Arr (strict)"("Number of Columns"=w189) -> ()  [unwired: 2 in, 2 out]
              n211 = property on="Voies EDWARDS" class="Arr (strict)"("Number of Columns"=w189) -> ()  [unwired: 2 in, 2 out]
              n212 = global write "Variable glob Edwards.vi" "Select Edwards"(w194) -> ()
              n213 = global write "Variable glob Edwards.vi" "Port RS232 Edwards"(w193) -> ()
              n214 = local write "Ports COM EDWARDS"(w193) -> ()
              n215 = global write "Variable glob Edwards.vi" "Select Grappes"(bool[] [] ("Sélect Grappes")) -> ()
              n216 = global write "Variable glob Edwards.vi" "Grappes"(string[][] [] ("Grappes")) -> ()
              n217 = local write "Noms jauges"(w191) -> ()
              n218 = global write "Variable glob Edwards.vi" "Voies Pres Edwards"(w192) -> ()
              n219 = local write "Voies EDWARDS"(w192) -> ()
              n220 = global write "Variable glob Edwards.vi" "Noms Edwards"(w191) -> ()
              n221 = property on="Noms jauges" class="Arr (strict)"("Number of Columns"=w189) -> ()  [unwired: 2 in, 2 out]
            }
            event "Ports COM EDWARDS", "Voies EDWARDS", "Noms jauges": Value Change {
              n222 = event-data() -> ()  [unwired: 1 in, 5 out]
              n223 = local read "Ports COM EDWARDS"() -> (w257:refnum<visa-resource-name>[])
              n224 = local read "Voies EDWARDS"() -> (w256:u8[][])
              n225 = local read "Noms jauges"() -> (w255:string[][])
              n226 = global write "Variable glob Edwards.vi" "Port RS232 Edwards"(w257) -> ()
              n227 = global write "Variable glob Edwards.vi" "Voies Pres Edwards"(w256) -> ()
              n228 = global write "Variable glob Edwards.vi" "Noms Edwards"(w255) -> ()
              n229 = Transpose 2D Array(2D array=w255) -> (transposed array=w254:string[][])
              n230 = local read "Grappes"() -> (w251:u16[][])
              n231 = control-ref of="Jauge Grappe"() -> (w252:refnum<vi>)
              n232 = for {
                tunnel: w254 -> [w266] mode=indexing
                shift-right: [w264] -> w250
                shift-left: string[] [] -> [w265]
                n233 = Build Array (concatenate)(w265, w266) -> (w264:string[])
              }
              n234 = for {
                tunnel: w251 -> [w260] mode=indexing
                tunnel: w250 -> [w259]
                tunnel: [w258] -> w249 mode=indexing
                n235 = for {
                  tunnel: w260 -> [w262] mode=indexing
                  tunnel: w259 -> [w263]
                  tunnel: [w261] -> w258 mode=indexing
                  n236 = Index Array(array=w263, index=w262) -> (element=w261:string)
                }
              }
              n237 = local read "Noms grappes"() -> (w248:string[])
              n238 = property class="Ring (strict)"(reference=w252, "Strings []"=w250) -> ()  [unwired: 1 in, 2 out]
              n239 = Insert Into Array(array=w249, index (col)=0 ("indice désactivé (col)"), new element=w248) -> (w246:string[][])  [unwired: 1 in]
              n240 = global write "Variable glob Edwards.vi" "Grappes"(w246) -> ()
            }
            event "Nombre de grappes": Value Change {
              n241 = event-data() -> ("OldVal"=w272:u8, "NewVal"=w271:u8)  [unwired: 1 in, 3 out]
              n242 = Equal To 0?(x=w271) -> (x = 0?=w273:bool)
              n243 = case shown="False" w273 {
                tunnel: w272 -> [w283 _]
                tunnel: w271 -> [w282 _]
                tunnel: [w281 string[] [] ("Noms jauges")] -> w268
                tunnel: [w278 u16[][] [] ("Grappes")] -> w270
                tunnel: [w276 bool[] [] ("Sélect Grappes")] -> w269
                tunnel: [w274 string[][] [] ("Grappes")] -> w267
                frame False {
                  n244 = Increment(x=w283) -> (x+1=w285:u8)
                  n245 = Subtract(x=w285, y=w282) -> (x-y=w284:u8)
                  n246 = global read "Variable glob Edwards.vi" "Select Grappes"() -> (w277:bool[])
                  n247 = local read "Noms grappes"() -> (w280:string[])
                  n248 = global read "Variable glob Edwards.vi" "Grappes"() -> (w275:string[][])
                  n249 = local read "Grappes"() -> (w279:u16[][])
                  n250 = case shown="0" w284 {
                    tunnel: w280 -> [w295 w307 w311]
                    tunnel: [w294 w306 w311] -> w281
                    tunnel: w282 -> [w291 _ _]
                    tunnel: w279 -> [w293 w298 w310]
                    tunnel: [w292 w296 w310] -> w278
                    tunnel: w277 -> [w290 w304 w309]
                    tunnel: [w289 w302 w309] -> w276
                    tunnel: w275 -> [w288 w301 w308]
                    tunnel: [w287 w299 w308] -> w274
                    frame 2 {
                      w286 = 1 ("longueur")
                      n251 = Delete From Array(array=w295, length=w286) -> (array with subset deleted=w294:string[])  [unwired: 1 in, 1 out]
                      n252 = Delete From Array(array=w290, length=w286) -> (array with subset deleted=w289:bool[])  [unwired: 1 in, 1 out]
                      n253 = Delete From Array(array=w288, length=w286) -> (array with subset deleted=w287:string[][])  [unwired: 2 in, 1 out]
                      n254 = Delete From Array(array=w293, length=w286, index (row)=w291) -> (array with subset deleted=w292:u16[][])  [unwired: 1 in, 1 out]
                    }
                    frame 0 {
                      n255 = Insert Into Array(array=w301, new element=string[] [] ("nouvel élément/sous-tableau")) -> (w299:string[][])  [unwired: 2 in]
                      n256 = Insert Into Array(array=w304, new element=TRUE ("nouvel élément/sous-tableau")) -> (w302:bool[])  [unwired: 1 in]
                      n257 = Insert Into Array(array=w298, new element=u16[] [] ("nouvel élément/sous-tableau")) -> (w296:u16[][])  [unwired: 2 in]
                      n258 = Insert Into Array(array=w307, new element="") -> (w306:string[])  [unwired: 1 in]
                    }
                    frame 1, Default {
                    }
                  }
                }
                frame True {
                }
              }
              n259 = property on="Grappes" class="Arr (strict)"("Number of Rows"=w271) -> ()  [unwired: 2 in, 2 out]
              n260 = property on="Noms grappes" class="Arr (strict)"("Number of Rows"=w271) -> ()  [unwired: 2 in, 2 out]
              n261 = local write "Noms grappes"(w268) -> ()
              n262 = global write "Variable glob Edwards.vi" "Select Grappes"(w269) -> ()
              n263 = local write "Grappes"(w270) -> ()
              n264 = global write "Variable glob Edwards.vi" "Grappes"(w267) -> ()
            }
            event "Grappes", "Noms grappes": Value Change {
              n265 = event-data() -> ()  [unwired: 1 in, 5 out]
              n266 = control-ref of="Jauge Grappe"() -> (w322:refnum<vi>)
              n267 = property class="Ring (strict)"(reference=w322) -> ("Strings []"=w321:string[])  [unwired: 1 in, 2 out]
              n268 = for {
                tunnel: "Grappes" -> [w325] mode=indexing
                tunnel: w321 -> [w324]
                tunnel: [w323] -> w319 mode=indexing
                n269 = for {
                  tunnel: w325 -> [w327] mode=indexing
                  tunnel: w324 -> [w328]
                  tunnel: [w326] -> w323 mode=indexing
                  n270 = Index Array(array=w328, index=w327) -> (element=w326:string)
                }
              }
              n271 = Insert Into Array(array=w319, index (col)=0 ("indice désactivé (col)"), new element="Noms grappes") -> (w316:string[][])  [unwired: 1 in]
              n272 = global write "Variable glob Edwards.vi" "Grappes"(w316) -> ()
            }
            event "Nb KELLER": Value Change {
              n273 = event-data() -> ("OldVal"=w334:i32, "NewVal"=w329:i32)  [unwired: 1 in, 3 out]
              n274 = Equal To 0?(x=w329) -> (x = 0?=w330:bool)
              n275 = case shown="False" w330 {
                tunnel: w334 -> [w342 _]
                tunnel: w329 -> [w341 _]
                tunnel: [w340 bool[] [] ("Sélection KELLER")] -> w333
                tunnel: [w338 i16[] [] ("Adresses KELLER")] -> w332
                tunnel: [w337 string[] [] ("Noms capteurs KELLER")] -> w331
                frame False {
                  n276 = Increment(x=w342) -> (x+1=w345:i32)
                  n277 = global read "Variable glob Keller.vi" "Selection KELLER"() -> (w339:bool[])
                  n278 = Subtract(x=w345, y=w341) -> (x-y=w343:i32)
                  n279 = Decrement(x=w341) -> (x-1=w344:i32)
                  n280 = case shown="2" w343 {
                    tunnel: "Adresses KELLER" -> [w352 w362 w364]
                    tunnel: [w351 w361 w364] -> w338
                    tunnel: "Noms capteurs KELLER" -> [w350 w360 w363]
                    tunnel: [w349 w359 w363] -> w337
                    tunnel: w344 -> [_ w355 _]
                    tunnel: w339 -> [w348 w356 w365]
                    tunnel: [w346 w353 w365] -> w340
                    frame 2 {
                      w347 = 1
                      # "1 capteur de moins"
                      n281 = Delete From Array(array=w352, length=w347) -> (array with subset deleted=w351:i16[])  [unwired: 1 in, 1 out]
                      n282 = Delete From Array(array=w350, length=w347) -> (array with subset deleted=w349:string[])  [unwired: 1 in, 1 out]
                      n283 = Delete From Array(array=w348, length=w347) -> (array with subset deleted=w346:bool[])  [unwired: 1 in, 1 out]
                    }
                    frame 0 {
                      # "1 capteur de plus"
                      n284 = call <vilib>:"Space Constant.vi"() -> ("String"=w357:string)
                      n285 = Insert Into Array(array=w362, index=w355, new element=0) -> (w361:i16[])
                      n286 = Insert Into Array(array=w356, index=w355, new element=TRUE) -> (w353:bool[])
                      n287 = Insert Into Array(array=w360, index=w355, new element=w357) -> (w359:string[])
                    }
                    frame 1, Default {
                      # "nombre de capteur\ninchangé"
                    }
                  }
                }
                frame True {
                }
              }
              n288 = property on="Adresses KELLER" class="Arr (strict)"("Number of Rows"=w329) -> ()  [unwired: 2 in, 2 out]
              n289 = property on="Noms capteurs KELLER" class="Arr (strict)"("Number of Rows"=w329) -> ()  [unwired: 2 in, 2 out]
              n290 = global write "Variable glob Keller.vi" "Selection KELLER"(w333) -> ()
              n291 = local write "Adresses KELLER"(w332) -> ()
              n292 = local write "Noms capteurs KELLER"(w331) -> ()
              n293 = global write "Variable glob Keller.vi" "Adresses KELLER"(w332) -> ()
              n294 = global write "Variable glob Keller.vi" "Noms KELLER"(w331) -> ()
            }
            event "Adresses KELLER", "Noms capteurs KELLER", "Port COM KELLER": Value Change {
              n295 = event-data() -> ()  [unwired: 1 in, 5 out]
              n296 = local read "Noms capteurs KELLER"() -> (w371:string[])
              n297 = local read "Adresses KELLER"() -> (w370:i16[])
              n298 = global write "Variable glob Keller.vi" "Port COM KELLER"("Port COM KELLER") -> ()
              n299 = global write "Variable glob Keller.vi" "Adresses KELLER"(w370) -> ()
              n300 = global write "Variable glob Keller.vi" "Noms KELLER"(w371) -> ()
            }
            event "Nombre de tâches thermocouples": Value Change {
              n301 = event-data() -> ("OldVal"=w379:u8, "NewVal"=w377:u8)  [unwired: 1 in, 1 out]
              n302 = Equal To 0?(x=w377) -> (x = 0?=w378:bool)
              n303 = case shown="False" w378 {
                tunnel: w379 -> [w386 _]
                tunnel: [w384 refnum<k21>[] [] ("Noms taches chassis Th")] -> w372
                tunnel: w377 -> [w383 _]
                frame False {
                  n304 = Increment(x=w386) -> (x+1=w387:u8)
                  n305 = Subtract(x=w387, y=w383) -> (x-y=w388:u8)
                  n306 = case shown="2" w388 {
                    tunnel: [w390 w392 w393] -> w384
                    tunnel: "Noms taches Th" -> [w391 w392 w394]
                    frame 0 {
                      n307 = call <vilib>:"Space Constant.vi"() -> ("String"=w389:string)
                      n308 = Insert Into Array(array=w391, new element=w389) -> (w390:refnum<k21>[])  [unwired: 1 in]
                    }
                    frame 1, Default {
                    }
                    frame 2 {
                      n309 = Delete From Array(array=w394, length=1 ("longueur")) -> (array with subset deleted=w393:refnum<k21>[])  [unwired: 1 in, 1 out]
                    }
                  }
                }
                frame True {
                }
              }
              n310 = global write "Variable glob Th.vi" "Nb de chassis Th"(w377) -> ()
              n311 = property on="Noms taches Th" class="Arr (strict)"("Number of Rows"=w377) -> ()  [unwired: 2 in, 2 out]
              n312 = property on="NB Th par tâche" class="Arr (strict)"("Number of Rows"=w377) -> ()  [unwired: 2 in, 2 out]
              n313 = local write "Noms taches Th"(w372) -> ()
              n314 = global read "Variable glob Th.vi" "Taches Th"() -> (w376:T9)
              n315 = Index Array(array=w376, index=0 ("indice")) -> (element=w374:T12)
              n316 = for {
                tunnel: w374 -> [w382]
                tunnel: [w381] -> w373 mode=indexing
                tunnel: w372 -> [w380] mode=indexing
                n317 = Bundle By Name(cluster=w382, "Nom tache Th"=w380) -> (w381:T12)
              }
              n318 = global write "Variable glob Th.vi" "Taches Th"(w373) -> ()
            }
            event "NB Th par tâche", "Noms taches Th": Value Change {
              n319 = event-data() -> ()  [unwired: 1 in, 5 out]
              n320 = local read "Noms taches Th"() -> (w404:refnum<k21>[])
              n321 = for {
                tunnel: w404 -> [w413] mode=indexing
                shift-right: [w413] -> _
                shift-left: refnum<k21> refnum ("Nom de la tache associée aux chassis") -> [w415]
                tunnel: [w414] -> w405
                stop <- w414 stop-if-true
                n322 = Equal?(x=w415, y=w413) -> (x = y?=w414:bool)
              }
              n323 = global read "Variable glob Th.vi" "Taches Th"() -> (w402:T9)
              n324 = case shown="True" w405 {
                tunnel: w404 -> [w410 _]
                tunnel: [w410 w411] -> w397
                frame False {
                }
                frame True {
                  w411 = refnum<k21>[] [] ("Noms taches chassis Th")
                  n325 = local write "Noms taches Th"(w411) -> ()
                  n326 = One Button Dialog(message="Vous ne pouvez pas sélectionner deux fois la même tâche") -> ()  [unwired: 1 in, 1 out]
                }
              }
              n327 = Index Array(array=w402, index=0 ("indice")) -> (element=w400:T12)
              n328 = for {
                tunnel: w400 -> [w409]
                tunnel: "NB Th par tâche" -> [w408] mode=indexing
                tunnel: [w407] -> w398 mode=indexing
                tunnel: w397 -> [w406] mode=indexing
                n329 = Bundle By Name(cluster=w409, "Nom tache Th"=w406, "Nb Th"=w408) -> (w407:T12)
              }
              n330 = global write "Variable glob Th.vi" "Taches Th"(w398) -> ()
            }
            event "Nombre de tâches Pt": Value Change {
              n331 = event-data() -> ("OldVal"=w423:u8, "NewVal"=w421:u8)  [unwired: 1 in, 3 out]
              n332 = Equal To 0?(x=w421) -> (x = 0?=w422:bool)
              n333 = case shown="False" w422 {
                tunnel: w423 -> [w430 _]
                tunnel: w421 -> [w428 _]
                tunnel: [w427 refnum<k21>[] [] ("Noms taches modules Pt")] -> w416
                frame False {
                  n334 = Increment(x=w430) -> (x+1=w431:u8)
                  n335 = Subtract(x=w431, y=w428) -> (x-y=w432:u8)
                  n336 = Decrement(x=w428) -> (x-1=w433:u8)
                  n337 = case shown="2" w432 {
                    tunnel: [w436 w438 w439] -> w427
                    tunnel: "Noms taches Pt" -> [w437 w438 w440]
                    tunnel: w433 -> [w435 _ _]
                    frame 0 {
                      n338 = call <vilib>:"Space Constant.vi"() -> ("String"=w434:string)
                      n339 = Insert Into Array(array=w437, index=w435, new element=w434) -> (w436:refnum<k21>[])
                    }
                    frame 1, Default {
                    }
                    frame 2 {
                      n340 = Delete From Array(array=w440, length=1 ("longueur")) -> (array with subset deleted=w439:refnum<k21>[])  [unwired: 1 in, 1 out]
                    }
                  }
                }
                frame True {
                }
              }
              n341 = global write "Variable glob Pt.vi" "Nb de chassis Pt"(w421) -> ()
              n342 = property on="Noms taches Pt" class="Arr (strict)"("Number of Rows"=w421) -> ()  [unwired: 2 in, 2 out]
              n343 = property on="NB Pt par tâche" class="Arr (strict)"("Number of Rows"=w421) -> ()  [unwired: 2 in, 2 out]
              n344 = global read "Variable glob Pt.vi" "Taches Pt 100"() -> (w420:T8)
              n345 = local write "Noms taches Pt"(w416) -> ()
              n346 = Index Array(array=w420, index=0 ("indice")) -> (element=w418:T13)
              n347 = for {
                tunnel: w418 -> [w426]
                tunnel: [w425] -> w417 mode=indexing
                tunnel: w416 -> [w424] mode=indexing
                n348 = Bundle By Name(cluster=w426, "Nom tache Pt"=w424) -> (w425:T13)
              }
              n349 = global write "Variable glob Pt.vi" "Taches Pt 100"(w417) -> ()
            }
            event "Noms taches Pt", "NB Pt par tâche": Value Change {
              n350 = event-data() -> ()  [unwired: 1 in, 2 out]
              n351 = local read "Noms taches Pt"() -> (w450:refnum<k21>[])
              n352 = for {
                tunnel: w450 -> [w460] mode=indexing
                shift-right: [w460] -> _
                shift-left: refnum<k21> refnum ("Nom de la tache associée aux modules") -> [w461]
                tunnel: [w459] -> w451
                stop <- w459 stop-if-true
                n353 = Equal?(x=w461, y=w460) -> (x = y?=w459:bool)
              }
              n354 = case shown="True" w451 {
                tunnel: w450 -> [w456 _]
                tunnel: [w456 w457] -> w443
                frame False {
                }
                frame True {
                  w457 = refnum<k21>[] [] ("Noms taches chassis Th")
                  n355 = local write "Noms taches Pt"(w457) -> ()
                  n356 = One Button Dialog(message="Vous ne pouvez pas sélectionner deux fois la même tâche") -> ()  [unwired: 1 in, 1 out]
                }
              }
              n357 = global read "Variable glob Pt.vi" "Taches Pt 100"() -> (w448:T8)
              n358 = Index Array(array=w448, index=0 ("indice")) -> (element=w446:T13)
              n359 = for {
                tunnel: w446 -> [w455]
                tunnel: "NB Pt par tâche" -> [w454] mode=indexing
                tunnel: [w453] -> w444 mode=indexing
                tunnel: w443 -> [w452] mode=indexing
                n360 = Bundle By Name(cluster=w455, "Nom tache Pt"=w452, "Nb Pt"=w454) -> (w453:T13)
              }
              n361 = global write "Variable glob Pt.vi" "Taches Pt 100"(w444) -> ()
            }
            event "Nb COM REG": Value Change {
              n362 = event-data() -> ("NewVal"=w473:u8, "OldVal"=w472:u8)  [unwired: 1 in]
              n363 = local read "Regulateurs EUROTHERM"() -> (w465:T3)
              n364 = local read "Ports COM REG"() -> (w470:refnum<visa-resource-name>[])
              n365 = Greater Or Equal?(x=w473, y=w472) -> (x >= y?=w471:bool)
              n366 = local read "Nb reg"() -> (w469:u8[])
              n367 = case shown="True" w471 {
                tunnel: w465 -> [w489 w500]
                tunnel: w470 -> [w488 w497]
                tunnel: w469 -> [w487 w494]
                tunnel: "Nb COM REG" -> [w486 w498]
                tunnel: [w485 w499] -> w464
                tunnel: [w484 w495] -> w466
                tunnel: [w483 w491] -> w467
                frame False {
                  n368 = Delete From Array(array=w489, index=w486) -> (array with subset deleted=w485:T3)  [unwired: 1 in, 1 out]
                  n369 = Delete From Array(array=w487, index=w486) -> (array with subset deleted=w483:u8[])  [unwired: 1 in, 1 out]
                  n370 = Delete From Array(array=w488, index=w486) -> (array with subset deleted=w484:refnum<visa-resource-name>[])  [unwired: 1 in, 1 out]
                }
                frame True {
                  n371 = Decrement(x=w498) -> (x-1=w492:u8)
                  n372 = Insert Into Array(array=w497, index=w492, new element=refnum<visa-resource-name> refnum ("nouvel élément/sous-tableau")) -> (w495:refnum<visa-resource-name>[])
                  n373 = Insert Into Array(array=w494, index=w492, new element=u8 0 ("nouvel élément/sous-tableau")) -> (w491:u8[])
                  n374 = Insert Into Array(array=w500, index=w492, new element=T5 {"Rég EUROTHERM 2"=[{"Nom"="", "Adresse"=0}]} ("nouvel élément/sous-tableau")) -> (w499:T3)
                }
              }
              n375 = for {
                tunnel: w464 -> [w479] mode=indexing
                tunnel: [w476] -> w462 mode=indexing
                tunnel: [w475] -> w463 mode=indexing
                n376 = Unbundle By Name(w479) -> ("1 COM reg"=w478:cluster{"Nom":string, "Adresse":u8}[])
                n377 = for {
                  tunnel: w478 -> [w482] mode=indexing
                  tunnel: [w481] -> w477 mode=indexing
                  tunnel: [w480] -> w474 mode=indexing
                  n378 = Unbundle By Name(w482) -> ("Nom"=w481:string, "Adresse"=w480:u8)
                }
                n379 = Bundle(w477) -> (w476:cluster{string[]})  [unwired: 1 in]
                n380 = Bundle(w474) -> (w475:cluster{u8[]})  [unwired: 1 in]
              }
              n381 = local write "Regulateurs EUROTHERM"(w464) -> ()
              n382 = global write "Variables glob EUROTHERM.vi" "Nb reg dispo"(w467) -> ()
              n383 = global write "Variables glob EUROTHERM.vi" "Ports COM REG dispo"(w466) -> ()
              n384 = local write "Nb reg"(w467) -> ()
              n385 = local write "Ports COM REG"(w466) -> ()
              n386 = property on="sur port COM :" class="Ring (strict)"("Strings []"=w466) -> ()  [unwired: 2 in, 2 out]
              n387 = global write "Variables glob EUROTHERM.vi" "Noms voies regs dispo"(w462) -> ()
              n388 = global write "Variables glob EUROTHERM.vi" "Adresses regs dispo"(w463) -> ()
            }
            event "Ports COM REG": Value Change {
              n389 = event-data() -> ()  [unwired: 1 in, 6 out]
              n390 = global write "Variables glob EUROTHERM.vi" "Ports COM REG dispo"("Ports COM REG") -> ()
              n391 = property on="sur port COM :" class="Ring (strict)"("Strings []"="Ports COM REG") -> ()  [unwired: 2 in, 2 out]
            }
            event "sur port COM :": Value Change {
              n392 = event-data() -> ("NewVal"=w504:u16)  [unwired: 1 in, 1 out]
              n393 = Build Array(w504, u16 0 ("élément")) -> (w502:u16[])
              n394 = property on="Regulateurs EUROTHERM" class="Arr (strict)"("Index Values"=w502) -> ()  [unwired: 2 in, 2 out]
            }
            event "Nb reg": Value Change {
              n395 = event-data() -> ("NewVal"=w518:u8[], "OldVal"=w521:u8[])  [unwired: 1 in]
              n396 = local read "Regulateurs EUROTHERM"() -> (w511:T3)
              n397 = Not Equal?(x=w518, y=w521) -> (x != y?=w520:bool[])
              n398 = Search 1D Array(1D array=w520, element=TRUE ("élément")) -> (index of element=w510:i32)  [unwired: 1 in]
              n399 = Index Array(array=w511, index=w510) -> (element=w512:T11)
              n400 = Index Array(array=w518, index=w510) -> (element=w517:u8)
              n401 = Unbundle By Name(w512) -> ("1 COM reg"=w514:cluster{"Nom":string, "Adresse":u8}[])
              n402 = Array Size(array=w514) -> (size(s)=w516:i32)
              n403 = Greater?(x=w517, y=w516) -> (0:w515:bool)
              n404 = case shown="False" w515 {
                tunnel: w514 -> [w533 w538]
                tunnel: [w531 w536] -> w513
                frame False {
                  # "1 reg de moins"
                  n405 = Array Size(array=w533) -> (size(s)=w534:i32)
                  n406 = Decrement(x=w534) -> (x-1=w532:i32)
                  n407 = Delete From Array(array=w533, length=1 ("longueur"), index=w532) -> (array with subset deleted=w531:cluster{"Nom":string, "Adresse":u8}[])  [unwired: 1 out]
                }
                frame True {
                  # "1 reg de plus"
                  n408 = Build Array (concatenate)(w538, cluster{"Nom":string, "Adresse":u8} {"Nom"="", "Adresse"=0}) -> (w536:cluster{"Nom":string, "Adresse":u8}[])
                }
              }
              n409 = Bundle By Name(cluster=w512, "1 COM reg"=w513) -> (w509:T11)
              n410 = Replace Array Subset(array=w511, new element=w509, index=w510) -> (w507:T3)
              n411 = local write "Regulateurs EUROTHERM"(w507) -> ()
              n412 = for {
                tunnel: w507 -> [w527] mode=indexing
                tunnel: [w525] -> w506 mode=indexing
                tunnel: [w522] -> w505 mode=indexing
                n413 = Unbundle By Name(w527) -> ("1 COM reg"=w526:cluster{"Nom":string, "Adresse":u8}[])
                n414 = for {
                  tunnel: w526 -> [w530] mode=indexing
                  tunnel: [w529] -> w524 mode=indexing
                  tunnel: [w528] -> w523 mode=indexing
                  n415 = Unbundle By Name(w530) -> ("Nom"=w529:string, "Adresse"=w528:u8)
                }
                n416 = Bundle(w524) -> (w525:cluster{string[]})  [unwired: 1 in]
                n417 = Bundle(w523) -> (w522:cluster{u8[]})  [unwired: 1 in]
              }
              n418 = global write "Variables glob EUROTHERM.vi" "Noms voies regs dispo"(w506) -> ()
              n419 = global write "Variables glob EUROTHERM.vi" "Adresses regs dispo"(w505) -> ()
              n420 = global write "Variables glob EUROTHERM.vi" "Nb reg dispo"("Nb reg") -> ()
            }
            event "Regulateurs EUROTHERM": Value Change {
              n421 = event-data() -> ("NewVal"=w540:T3)  [unwired: 1 in, 1 out]
              n422 = for {
                tunnel: w540 -> [w550] mode=indexing
                tunnel: [w547] -> w542 mode=indexing
                tunnel: [w545] -> w541 mode=indexing
                tunnel: [w543] -> w539 mode=indexing
                n423 = Unbundle By Name(w550) -> ("1 COM reg"=w549:cluster{"Nom":string, "Adresse":u8}[])
                n424 = for {
                  tunnel: w549 -> [w554] mode=indexing
                  tunnel: [w553] -> w548 mode=indexing
                  tunnel: [w552] -> w546 mode=indexing
                  tunnel: [TRUE] -> w544 mode=indexing
                  n425 = Unbundle By Name(w554) -> ("Nom"=w553:string, "Adresse"=w552:u8)
                }
                n426 = Bundle(w546) -> (w545:cluster{u8[]})  [unwired: 1 in]
                n427 = Bundle(w544) -> (w543:cluster{bool[]})  [unwired: 1 in]
                n428 = Bundle(w548) -> (w547:cluster{string[]})  [unwired: 1 in]
              }
              n429 = global write "Variables glob EUROTHERM.vi" "Select regs acqui"(w539) -> ()
              n430 = global write "Variables glob EUROTHERM.vi" "Noms voies regs dispo"(w542) -> ()
              n431 = global write "Variables glob EUROTHERM.vi" "Adresses regs dispo"(w541) -> ()
            }
            event "Nb compteurs": Value Change {
              n432 = event-data() -> ()  [unwired: 1 in, 6 out]
              n433 = Equal To 0?(x="Nb compteurs") -> (x = 0?=w558:bool)
              n434 = Select(t=T6."Disabled and Grayed Out" ("Désactivé"), s=w558, f=T6."Enabled" ("Désactivé")) -> (s? t:f=w555:T6)
              n435 = property on="Nom tache compteurs" class="DAQmxName (strict)"("DisabledEnum"=w555) -> ()  [unwired: 2 in, 2 out]
              n436 = property on="Noms des compteurs" class="Arr (strict)"("Number of Rows"="Nb compteurs", "DisabledEnum"=w555) -> ()  [unwired: 2 in, 2 out]
            }
            event "Nom tache compteurs", "Noms des compteurs": Value Change {
              n437 = event-data() -> ()  [unwired: 1 in, 6 out]
              n438 = global read "Variable globale compteurs.vi" "Tache Compteurs"() -> (w574:T10)
              n439 = Unbundle By Name(w574) -> ("Selection"=w570:bool[], "Init compteurs"=w565:dbl[])
              n440 = Array Size(array="Noms des compteurs") -> (size(s)=w563:i32)
              n441 = Array Size(array=w565) -> (size(s)=w567:i32)
              n442 = Array Size(array=w570) -> (size(s)=w572:i32)
              n443 = Not Equal?(x=w563, y=w567) -> (x != y?=w566:bool)
              n444 = Initialize Array(0.0, w563) -> (w564:dbl[])
              n445 = Initialize Array(TRUE, w563) -> (w568:bool[])
              n446 = Not Equal?(x=w563, y=w572) -> (x != y?=w571:bool)
              n447 = Select(t=w564, s=w566, f=w565) -> (s? t:f=w560:dbl[])
              n448 = Select(t=w568, s=w571, f=w570) -> (s? t:f=w561:bool[])
              n449 = Bundle By Name(cluster=w574, "Nom tache compteurs"="Nom tache compteurs", "Noms des compteurs"="Noms des compteurs", "Selection"=w561, "Init compteurs"=w560) -> (w576:T10)
              n450 = global write "Variable globale compteurs.vi" "Tache Compteurs"(w576) -> ()
            }
            event "annuler": Value Change {
              n451 = event-data() -> ()  [unwired: 1 in, 6 out]
            }
            event "stop": Value Change {
              # "Vérification qu'il n'y a pas deux COM identiques"
              n452 = event-data() -> ()  [unwired: 1 in, 2 out]
              n453 = stacked-sequence {
                seq-local: [w596 _ _ _ _] -> [_ w601 w608 _ _]
                seq-local: [_ w603 _ _ _] -> [_ _ _ _ _]
                seq-local: [_ _ w609 _ _] -> [_ _ _ w617 _]
                tunnel: [_ _ _ w614 _] -> w594
                frame #0 {
                  n454 = local read "Nb LEYBOLD"() -> (w598:i8)
                  n455 = local read "Ports COM LEYBOLDS"() -> (w600:refnum<visa-resource-name>[])
                  n456 = Equal To 0?(x=w598) -> (x = 0?=w599:bool)
                  n457 = Select(t=refnum<visa-resource-name>[] [] ("cas vrai"), s=w599, f=w600) -> (s? t:f=w596:refnum<visa-resource-name>[])
                }
                frame #1 {
                  n458 = local read "Nb EDWARDS"() -> (w606:i8)
                  n459 = local read "Ports COM EDWARDS"() -> (w605:refnum<visa-resource-name>[])
                  n460 = Equal To 0?(x=w606) -> (x = 0?=w604:bool)
                  n461 = Build Array (concatenate)(w601, w605) -> (w602:refnum<visa-resource-name>[])
                  n462 = Select(t=w601, s=w604, f=w602) -> (s? t:f=w603:refnum<visa-resource-name>[])
                }
                frame #2 {
                  n463 = local read "Port COM KELLER"() -> (w611:refnum<visa-resource-name>)
                  n464 = local read "Nb KELLER"() -> (w612:i32)
                  n465 = Equal To 0?(x=w612) -> (x = 0?=w610:bool)
                  n466 = Build Array (concatenate)(w608, w611) -> (w607:refnum<visa-resource-name>[])
                  n467 = Select(t=w608, s=w610, f=w607) -> (s? t:f=w609:refnum<visa-resource-name>[])
                }
                frame #3 {
                  n468 = local read "Nb reg"() -> (w619:u8[])
                  n469 = local read "Ports COM REG"() -> (w616:refnum<visa-resource-name>[])
                  n470 = Add Array Elements(numeric array=w619) -> (sum=w613:u8)
                  n471 = Equal To 0?(x=w613) -> (x = 0?=w618:bool)
                  n472 = Build Array (concatenate)(w617, w616) -> (w615:refnum<visa-resource-name>[])
                  n473 = Select(t=w617, s=w618, f=w615) -> (s? t:f=w614:refnum<visa-resource-name>[])
                }
                frame #4 {
                  n474 = global write "Variable glob Edwards.vi" "Seuil Jauge"("Seuil Jauge") -> ()
                }
              }
              n475 = global read "Variable globale compteurs.vi" "Tache Compteurs"() -> (w582:T10)
              n476 = global write "Variable globale compteurs.vi" "Temps débit"(u16 1 ("Temps débit")) -> ()
              n477 = Unbundle By Name(w582) -> ("Noms des compteurs"=w589:string[], "Selection"=w587:bool[], "Init compteurs"=w584:dbl[])
              n478 = local read "Nb compteurs"() -> (w583:u8)
              n479 = Sort 1D Array(array=w594) -> (sorted array=w595:refnum<visa-resource-name>[])
              n480 = for {
                tunnel: w595 -> [w627] mode=indexing
                shift-right: [w627] -> _
                shift-left: refnum<visa-resource-name> refnum ("x") -> [w628]
                shift-right: [w625] -> _
                shift-left: FALSE -> [w626]
                n481 = Equal?(x=w627, y=w628) -> (x = y?=w623:bool)
                n482 = Equal?(x=refnum<visa-resource-name> refnum, y=w627) -> (x = y?=w622:bool)
                n483 = Or(x=w622, y=w623) -> (x .or. y?=w621:bool)
                n484 = case shown="True" w621 {
                  tunnel: w626 -> [w629 _]
                  tunnel: [w629 TRUE] -> w625
                  frame False {
                  }
                  frame True {
                    n485 = One Button Dialog(message="ERREUR SUR PORT COM :\nDEUX PORTS SONT IDENTIQUES OU UN PORT N'EST PAS RENSEIGNÉ.\nCETTE CONFIGURATION NE PEUT ÊTRE ENREGISTRÉE.") -> ()  [unwired: 1 in, 1 out]
                  }
                }
              }
              n486 = Delete From Array(array=w589, length=w583, index=0 ("indice")) -> (deleted portion=w581:string[])  [unwired: 1 out]
              n487 = Delete From Array(array=w587, length=w583, index=0 ("indice")) -> (deleted portion=w580:bool[])  [unwired: 1 out]
              n488 = Delete From Array(array=w584, length=w583, index=0 ("indice")) -> (deleted portion=w579:dbl[])  [unwired: 1 out]
              n489 = Bundle By Name(cluster=w582, "Noms des compteurs"=w581, "Selection"=w580, "Init compteurs"=w579) -> (w578:T10)
              n490 = global write "Variable globale compteurs.vi" "Tache Compteurs"(w578) -> ()
            }
          }
        }
        n491 = Select(t=Enum_conf_1."annule" ("Énum"), s=w131, f=Enum_conf_1."enregistrer fichier config" ("Énum")) -> (s? t:f=w128:T4)
      }
      frame "enregistrer fichier config" {
        # "écriture des paramètres de config\n- dans le fichier contenant le nom de la cuve\n- dans le fichier de base (qui sera utilisé pour les acquisitions)"
        n492 = Build Path(base path=path "C:/LABVIEW/PRES+TEMP+REG dernière version/Configurations", name or relative path="config acqui.ini") -> (appended path=w652:path)
        n493 = call <vilib>:"Open Config Data.vi"("create file if necessary (T)"=TRUE, "configuration file path"=w652) -> ("error out"=w649:errorcluster, "refnum"=w650:T7)  [unwired: 7 in, 1 out]
        n494 = call "Ecrire config gene.vi"("error in (no error)"=w649, "refnum"=w650) -> ("error out"=w645:errorcluster, "refnum out"=w637:T7)
        n495 = call "Ecrire config LEYBOLD.vi"("error in (no error)"=w645, "refnum"=w637) -> ("error out"=w646:errorcluster, "refnum out"=w638:T7)
        n496 = call "Ecrire config EDWARDS.vi"("error in (no error)"=w646, "refnum"=w638) -> ("error out"=w640:errorcluster, "refnum out"=w639:T7)
        n497 = call "Ecrire config KELLER.vi"("error in (no error)"=w640, "refnum"=w639) -> ("error out"=w642:errorcluster, "refnum out"=w641:T7)
        n498 = call "Ecrire config Th.vi"("error in (no error)"=w642, "refnum"=w641) -> ("error out"=w644:errorcluster, "refnum out"=w643:T7)
        n499 = call "Ecrire config.vi"("error in (no error)"=w644, "refnum"=w643) -> ("error out"=w648:errorcluster, "refnum out"=w647:T7)
        n500 = call "Ecrire config REG.vi"("error in (no error) 2"=w648, "refnum 2"=w647) -> ("error out"=w635:errorcluster, "refnum out"=w636:T7)
        n501 = call "Ecrire config compteurs.vi"("error in (no error)"=w635, "refnum"=w636) -> ("error out"=w633:errorcluster, "refnum out"=w634:T7)
        n502 = call <vilib>:"Close Config Data.vi"("error in (no error)"=w633, "refnum"=w634) -> ()  [unwired: 8 in, 2 out]
      }
      frame "annule" {
        n503 = call "Afficher un message à l'utilisateur"("Message"="Aucune modification n'est enregistrée") -> ()  [unwired: 9 in, 2 out]
      }
      frame "fin" {
        n504 = disable-structure shown="Activé" {
          frame Enabled {
            n505 = call "Chemin VI actuel (VI or exe).vi"() -> ("Full Path to VI or executable"=w660:path)  [unwired: 14 in, 1 out]
            n506 = Open VI Reference(vi path=w660) -> (vi reference=w663:refnum<vi>, error out=w662:errorcluster)  [unwired: 5 in]
            n507 = invoke class="VI" method="FP.Close"(reference=w663, error in=w662) -> (error out=w661:errorcluster)  [unwired: 1 in, 2 out]
            n508 = call <vilib>:"Clear Errors.vi"("error in (no error)"=w661) -> ()  [unwired: 5 in, 2 out]
          }
          frame Disabled {
          }
        }
        n509 = Request Deallocation(TRUE ("flag")) -> ()
      }
    }
  }
